vi "VIH HelpGen - Palette - Read Reference to Dynamic Palette.vi"(10 "Get Items (F)":bool, 11 "Palette Path":path) -> (0 "Data available":bool, 1 "palette data":T1={"display name"="", "view format"=0, "palette width"=4, "items"=[], "256 color icon"=bytes[0], "B&W color icon"=bytes[0], "help information"={"help tag"="", "help file path "=path ""}, "palette description"="", "synchronize information"={"synchronize with directory"=FALSE, "synchronize directory path"=path ""}} {"view format" items=["Icons", "Text", "Icons and Text"]})   [LabVIEW 2014]
doc: "::: VI Helpeks :::\nCopyright (c) 2000-2026 Konstantin Shifershteyn. All rights reserved."
uses:
  <vilib>/Palette API/Palette Menu/Public Type Define/Palette Data.ctl
  <vilib>/Palette API/Palette Menu/Public Type Define/View Format.ctl
  <vilib>/Palette API/Palette Menu/Public Type Define/Items.ctl
  <vilib>/Palette API/Palette Menu/Public Type Define/Item.ctl
  <vilib>/Palette API/Palette Menu/Public Type Define/Help Info.ctl
  <vilib>/Palette API/Palette Menu/Public Type Define/Synchronize Info.ctl
  <vilib>/Palette API/Palette Menu/Palette Menu.lvlib
panel:
  in  "DefIcon - Default Palette":picture
  # "VI Helpeks\nCopyright (c) 2012-2026 Konstantin Shifershteyn"
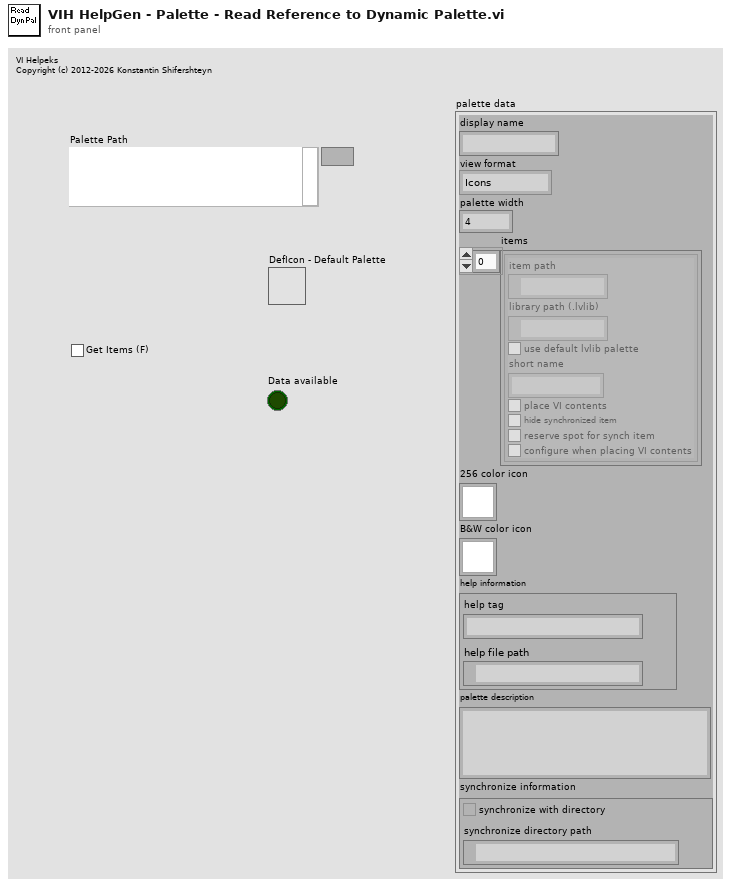
[diagram p1: front panel]
types:
  T1 = typedef "Palette Menu.lvlib/Palette Data.ctl" = cluster{"display name":string, "view format":T2, "palette width":i16, "items":T3, "256 color icon":picture, "B&W color icon":picture, "help information":T5, "palette description":string, "synchronize information":T6}
  T2 = typedef "Palette Menu.lvlib/View Format.ctl" = u16
  T3 = typedef "Palette Menu.lvlib/Items.ctl" = T4[]
  T4 = typedef "Palette Menu.lvlib/Item.ctl" = cluster{"item path":path, "library path (.lvlib)":path, "use default lvlib palette":bool, "short name":string, "place VI contents":bool, "hide synchronized item":bool, "reserve spot for synch item":bool, "configure when placing VI contents":bool}
  T5 = typedef "Palette Menu.lvlib/Help Info.ctl" = cluster{"help tag":string, "help file path ":path}
  T6 = typedef "Palette Menu.lvlib/Synchronize Info.ctl" = cluster{"synchronize with directory":bool, "synchronize directory path":path}
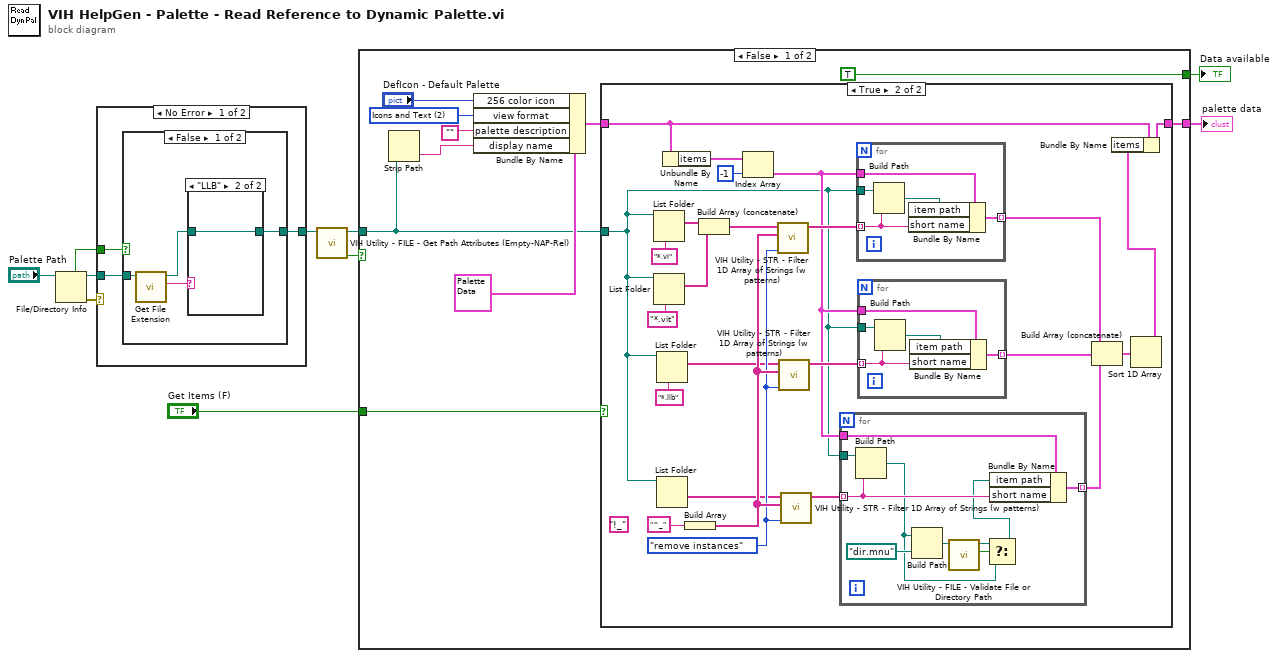
[diagram p0: block diagram]
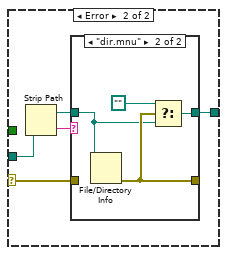
[diagram p6: hidden frame]
diagram:
  n1 = File/Directory Info(path="Palette Path") -> (path out=w7:path, directory=w8:bool, error out=w9:errorcluster)  [unwired: 1 in, 4 out]
  n2 = case shown="No Error" w9 {
    selector: w9 -> [_ w21]
    tunnel: w8 -> [w13 _]
    tunnel: w7 -> [w12 w24]
    tunnel: [w11 w20] -> w6
    frame No Error {
      n3 = case shown="False" w13 {
        tunnel: w12 -> [w17 w19]
        tunnel: [w14 w19] -> w11
        frame False {
          n4 = call <vilib>:"Get File Extension.vi"("file"=w17) -> ("lowercase file extension"=w16:string, "dup file"=w15:path)  [unwired: 7 in, 2 out]
          n5 = case shown="\"LLB\"" w16 {
            tunnel: w15 -> [_ w18]
            tunnel: [_ w18] -> w14
            frame Default {
            }
            frame "LLB" {
            }
          }
        }
        frame True {
        }
      }
    }
    frame Error {
      n6 = Strip Path(path=w24) -> (stripped path=w22:path, name=w23:string)
      n7 = case shown="\"dir.mnu\"" w23 {
        tunnel: w22 -> [_ w27]
        tunnel: [w25 w29] -> _
        tunnel: w21 -> [w25 _]
        tunnel: [_ w28] -> w20
        frame Default {
        }
        frame "dir.mnu" {
          n8 = File/Directory Info(path=w27) -> (error out=w29:errorcluster)  [unwired: 1 in, 6 out]
          n9 = Select(t=path "", s=w29, f=w27) -> (s? t:f=w28:path)
        }
      }
    }
  }
  n10 = call "VIH Utility - FILE - Get Path Attributes (Empty-NAP-Rel).vi"("Path"=w6) -> ("Not A Path or Empty path"=w5:bool, "dup Path"=w4:path)  [unwired: 6 in, 3 out]
  n11 = case shown="False" w5 {
    tunnel: w4 -> [w33 _]
    tunnel: "Get Items (F)" -> [w34 _]
    tunnel: [w31 _] -> w2
    tunnel: [TRUE _] -> w1
    frame False {
      w38 = T2 2 items=["Icons", "Text", "Icons and Text"] ("view format")
      n12 = Strip Path(path=w33) -> (name=w35:string)  [unwired: 1 out]
      n13 = Bundle By Name(cluster=T1 {"display name"="", "view format"=0, "palette width"=4, "items"=[], "256 color icon"=bytes[0], "B&W color icon"=bytes[0], "help information"={"help tag"="", "help file path "=path ""}, "palette description"="", "synchronize information"={"synchronize with directory"=FALSE, "synchronize directory path"=path ""}} ("palette data"), "256 color icon"="DefIcon - Default Palette", "view format"=w38, "palette description"="", "display name"=w35) -> (w32:T1)
      n14 = case shown="True" w34 {
        tunnel: w33 -> [_ w48]
        tunnel: w32 -> [w40 w43]
        tunnel: [w40 w42] -> w31
        frame False {
        }
        frame True {
          (unwired) "!_"
          w55 = enum16{"keep instances", "remove instances"}."remove instances" ("Action (keep instances)")
          n15 = List Folder(path=w48, pattern="*.vi") -> (filenames=w62:string[])  [unwired: 2 in, 3 out]
          n16 = List Folder(path=w48, pattern="*.vit") -> (filenames=w61:string[])  [unwired: 2 in, 3 out]
          n17 = List Folder(path=w48, pattern="*.llb") -> (filenames=w53:string[])  [unwired: 2 in, 3 out]
          n18 = List Folder(path=w48) -> (folder names=w52:string[])  [unwired: 3 in, 3 out]
          n19 = Unbundle By Name(w43) -> ("items"=w59:T3)
          n20 = Build Array("^_") -> (w56:string[])
          n21 = Build Array (concatenate)(w62, w61) -> (w60:string[])
          n22 = Index Array(array=w59, index=-1) -> (element=w49:T4)
          n23 = call "VIH Utility - STR - Filter 1D Array of Strings (w patterns).vi"("Action (keep instances)"=w55, "Regular expressions"=w56, "Array in"=w60) -> ("Array out"=w57:string[])  [unwired: 8 in]
          n24 = call "VIH Utility - STR - Filter 1D Array of Strings (w patterns).vi"("Action (keep instances)"=w55, "Regular expressions"=w56, "Array in"=w53) -> ("Array out"=w51:string[])  [unwired: 8 in]
          n25 = call "VIH Utility - STR - Filter 1D Array of Strings (w patterns).vi"("Action (keep instances)"=w55, "Regular expressions"=w56, "Array in"=w52) -> ("Array out"=w50:string[])  [unwired: 8 in]
          n26 = for {
            tunnel: w49 -> [w75]
            tunnel: w50 -> [w72] mode=indexing
            tunnel: w48 -> [w74]
            tunnel: [w73] -> w45 mode=indexing
            n27 = Build Path(base path=w74, name or relative path=w72) -> (appended path=w67:path)
            n28 = Build Path(base path=w67, name or relative path=path "dir.mnu") -> (appended path=w70:path)
            n29 = call "VIH Utility - FILE - Validate File or Directory Path.vi"("Path"=w70) -> ("file"=w69:bool, "dup Path"=w68:path)  [unwired: 6 in, 3 out]
            n30 = Select(t=w68, s=w69, f=w67) -> (s? t:f=w66:path)
            n31 = Bundle By Name(cluster=w75, "item path"=w66, "short name"=w72) -> (w73:T4)
          }
          n32 = for {
            tunnel: w49 -> [w85]
            tunnel: w57 -> [w84] mode=indexing
            tunnel: w48 -> [w82]
            tunnel: [w81] -> w46 mode=indexing
            n33 = Build Path(base path=w82, name or relative path=w84) -> (appended path=w83:path)
            n34 = Bundle By Name(cluster=w85, "item path"=w83, "short name"=w84) -> (w81:T4)
          }
          n35 = for {
            tunnel: w49 -> [w80]
            tunnel: w51 -> [w79] mode=indexing
            tunnel: w48 -> [w77]
            tunnel: [w76] -> w47 mode=indexing
            n36 = Build Path(base path=w77, name or relative path=w79) -> (appended path=w78:path)
            n37 = Bundle By Name(cluster=w80, "item path"=w78, "short name"=w79) -> (w76:T4)
          }
          n38 = Build Array (concatenate)(w46, w47, w45) -> (w44:T4[])
          n39 = Sort 1D Array(array=w44) -> (sorted array=w41:T4[])
          n40 = Bundle By Name(cluster=w43, "items"=w41) -> (w42:T1)
        }
      }
    }
    frame True {
    }
  }
  "palette data" <- w2
  "Data available" <- w1
